vi "RDV-sortData.vi"(8 "error in (no error)":errorcluster, 11 "RDV-Reflection_Data_viewer in":refnum<class "RDV-Reflection_Data_viewer.lvclass">) -> (0 "error out":errorcluster, 3 "RDV-Reflection_Data_viewer out":refnum<class "RDV-Reflection_Data_viewer.lvclass">)   [LabVIEW 2020, in "RDV-Reflection_Data_viewer.lvclass"]
doc: "Sorts the data in the viewer's map into the plot data."
uses:
  RDV-Reflection_Data_viewer.lvclass
  RDV-Reflection_Data_viewer.lvclass/RDV-Reflection_Data_viewer.ctl
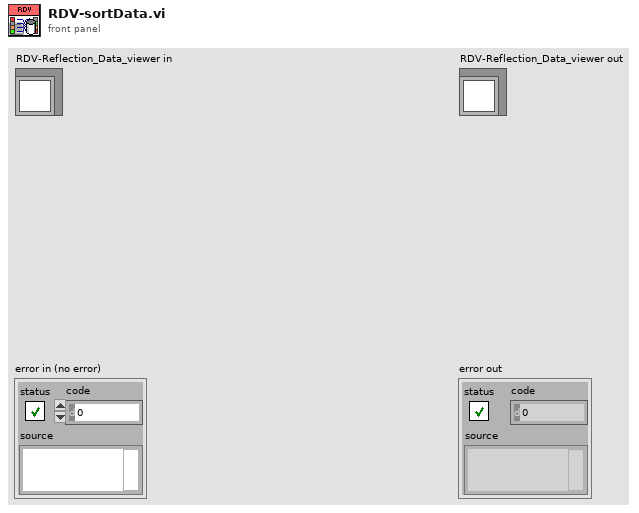
[diagram p1: front panel]
types:
  T1 = typedef "RDV-Reflection_Data_viewer.lvclass/RDV-DATA_MAP.ctl" = map{string, T2}
  T2 = typedef "RDV-Reflection_Data_viewer.lvclass/RDV-DATA_MAP_CLUST.ctl" = cluster{"filename w/ ext":string, "Common Format":T3}
  T3 = typedef "RFH-Reflection_File_Handler.lvlib/RFH-common_data_format.ctl" = cluster{"Frequency":dbl[], "Reflection'":dbl[], "Reflection''":dbl[], "Permativity'":dbl[], "Permativity''":dbl[], "Conductivity":dbl[], "Loss Tangent":dbl[], "Resistance":dbl[], "Reactance":dbl[]}
  T4 = cluster{"Frequency":dbl[], "Permativity''":dbl[]}
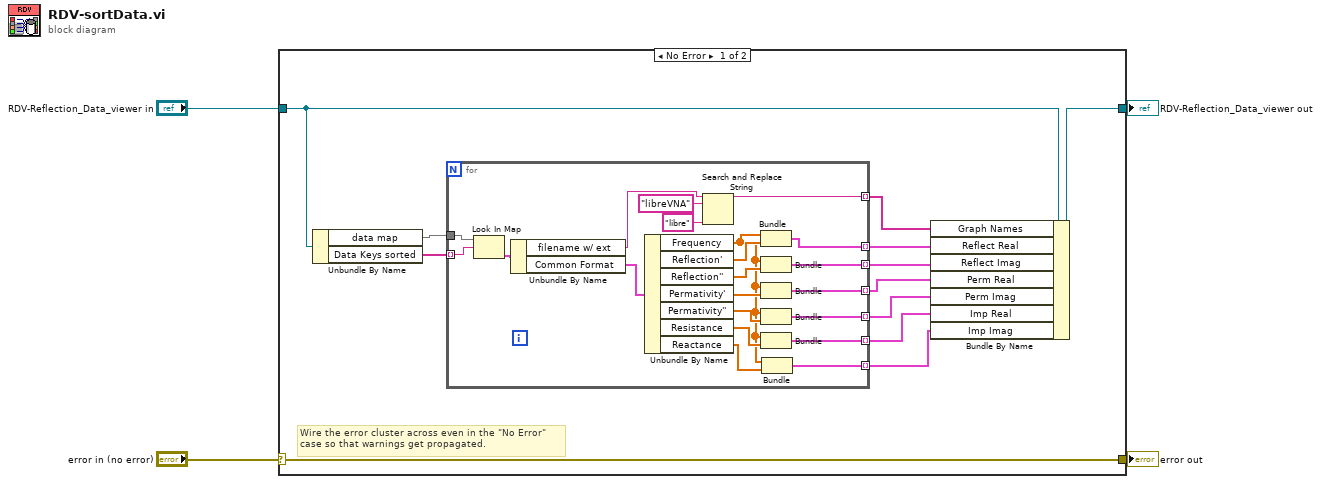
[diagram p0: block diagram]
diagram:
  n1 = case shown="No Error" "error in (no error)" {
    selector: "error in (no error)" -> [w16 w39]
    tunnel: [w16 w39] -> w3
    tunnel: [w13 w38] -> w1
    tunnel: "RDV-Reflection_Data_viewer in" -> [w15 w38]
    frame No Error {
      # "Wire the error cluster across even in the \"No Error\"\ncase so that warnings get propagated."
      n2 = Unbundle By Name(w15) -> ("data map"=w5:T1, "Data Keys sorted"=w14:string[])
      n3 = for {
        tunnel: [w35] -> w11 mode=indexing
        tunnel: [w34] -> w10 mode=indexing
        tunnel: w14 -> [w20] mode=indexing
        tunnel: [w31] -> w12 mode=indexing
        tunnel: [w28] -> w9 mode=indexing
        tunnel: [w24] -> w8 mode=indexing
        tunnel: [w23] -> w7 mode=indexing
        tunnel: [w22] -> w6 mode=indexing
        tunnel: w5 -> [w21]
        n4 = Look In Map(map=w21, key=w20) -> (value=w19:T2)  [unwired: 1 in, 1 out]
        n5 = Unbundle By Name(w19) -> ("filename w/ ext"=w17:string, "Common Format"=w18:T3)
        n6 = Unbundle By Name(w18) -> ("Frequency"=w25:dbl[], "Reflection'"=w37:dbl[], "Reflection''"=w36:dbl[], "Permativity'"=w30:dbl[], "Permativity''"=w29:dbl[], "Resistance"=w27:dbl[], "Reactance"=w26:dbl[])
        n7 = Search and Replace String(input string=w17, search string="libreVNA", replace string="libre" ("replace string (\"\")")) -> (result string=w31:string)  [unwired: 5 in, 3 out]
        n8 = Bundle("Frequency"=w25, "Reflection'"=w37) -> (w35:cluster{"Frequency":dbl[], "Reflection'":dbl[]})  [unwired: 1 in]
        n9 = Bundle("Frequency"=w25, "Reflection''"=w36) -> (w34:cluster{"Frequency":dbl[], "Reflection''":dbl[]})  [unwired: 1 in]
        n10 = Bundle("Frequency"=w25, "Permativity'"=w30) -> (w28:cluster{"Frequency":dbl[], "Permativity'":dbl[]})  [unwired: 1 in]
        n11 = Bundle("Frequency"=w25, "Permativity''"=w29) -> (w24:T4)  [unwired: 1 in]
        n12 = Bundle("Frequency"=w25, "Resistance"=w27) -> (w23:cluster{"Frequency":dbl[], "Resistance":dbl[]})  [unwired: 1 in]
        n13 = Bundle("Frequency"=w25, "Reactance"=w26) -> (w22:cluster{"Frequency":dbl[], "Reactance":dbl[]})  [unwired: 1 in]
      }
      n14 = Bundle By Name(cluster=w15, "Graph Names"=w12, "Reflect Real"=w11, "Reflect Imag"=w10, "Perm Real"=w9, "Perm Imag"=w8, "Imp Real"=w7, "Imp Imag"=w6) -> (w13:refnum<class "RDV-Reflection_Data_viewer.lvclass">)
    }
    frame Error {
    }
  }
  "error out" <- w3
  "RDV-Reflection_Data_viewer out" <- w1
